vi "test resource blob.vi"(8 "error in (no error)":errorcluster) -> (0 "error out":errorcluster, 3 "body":string)   [LabVIEW 2020, in "MCP Server tests.lvlib"]
doc: "resources/read of a binary file (image/png) must return blob: the Base64 encoding of the exact bytes of the file, as a plain JSON string."
uses:
  MCP Server tests.lvlib
  <vilib>/JDP Science/JSONtext/Next JSON Value.vi
  <vilib>/JDP Science/JSONtext/String Subset.vi
  <vilib>/JDP Science/JSONtext/Parsing/Advance past next JSON Value (inlined COPY).vi
  <vilib>/JDP Science/JSONtext/Parsing/Advance past whitespace.vi
  <vilib>/JDP Science/JSONtext/Parsing/Advance past String.vi
  <vilib>/JDP Science/JSONtext/Parsing/Advance past Number.vi
  <vilib>/JDP Science/JSONtext/Parsing/Advance past Line Ending.vi
  <vilib>/JDP Science/JSONtext/Parsing/Parse Full Path or Item Name.vi
  <vilib>/JDP Science/JSONtext/Parsing/Advance past Array.vi
  <vilib>/JDP Science/JSONtext/Parsing/Advance past Object.vi
  <vilib>/JDP Science/JSONtext/support/Error Cluster From Code.vi
  <vilib>/JDP Science/JSONtext/Offset/Find Item Locations by Path.vi
  <vilib>/addons/_JKI Toolkits/Caraya/classes/Test/Test.lvclass
  <vilib>/JDP Science/JSONtext/JSONtext.lvlib
  <vilib>/JDP Science/JDP Science Common Utilities/Base64/Base64 Support.lvlib
  <vilib>/addons/_JKI Toolkits/Caraya/classes/Assert/Assert.lvclass
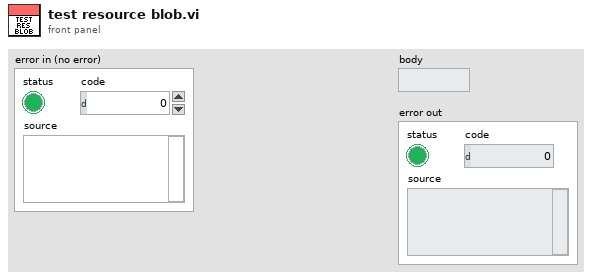
[diagram p1: front panel]
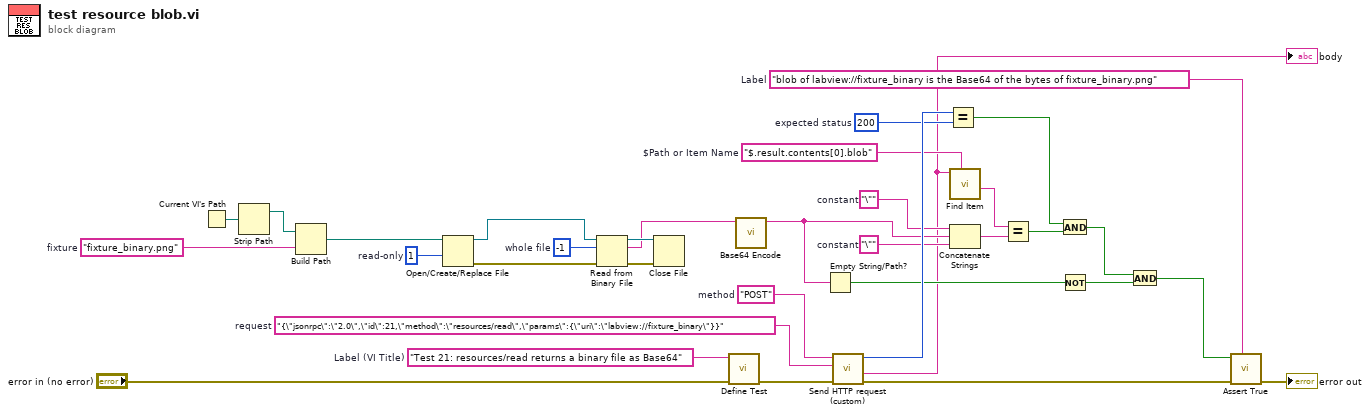
[diagram p0: block diagram]
diagram:
  w3 = "blob of labview://fixture_binary is the Base64 of the bytes of fixture_binary.png"  # Label
  w14 = "\""  # constant
  w15 = "\""  # constant
  w20 = -1  # whole file
  w22 = u32 1  # read-only
  w24 = "fixture_binary.png"  # fixture
  w27 = "$.result.contents[0].blob"  # $Path or Item Name
  w28 = 200  # expected status
  w31 = "{\"jsonrpc\":\"2.0\",\"id\":21,\"method\":\"resources/read\",\"params\":{\"uri\":\"labview://fixture_binary\"}}"  # request
  w32 = "POST"  # method
  w34 = "Test 21: resources/read returns a binary file as Base64"  # Label (VI Title)
  n1 = Current VI's Path() -> (path=w26:path)
  n2 = Strip Path(path=w26) -> (stripped path=w25:path)  [unwired: 1 out]
  n3 = Build Path(base path=w25, name or relative path=w24) -> (appended path=w23:path)
  n4 = Open/Create/Replace File(file path (use dialog)=w23, access (0:read/write)=w22) -> (refnum out=w21:refnum<file>, error out=w19:errorcluster)  [unwired: 4 in, 1 out]
  n5 = Read from Binary File(8:w19, 10:w20, 11:w21) -> (0:w17:errorcluster, 2:w16:string, 3:w18:refnum<file>)  [unwired: 3 in, 1 out]
  n6 = Close File(refnum=w18, error in=w17) -> ()  [unwired: 2 out]
  n7 = call <vilib>:"Define Test.vi"("error in (no error)"="error in (no error)", "Label (VI Title)"=w34) -> ("error out"=w30:errorcluster)  [unwired: 8 in, 1 out]
  n8 = call <vilib>:"Base64 Encode.vi"("String to Encode"=w16) -> ("Base64 Encoded"=w11:string)  [unwired: 10 in]
  n9 = Empty String/Path?(string/path=w11) -> (empty?=w10:bool)
  n10 = call "Send HTTP request (custom).vi"("error in (no error)"=w30, "request"=w31, "method"=w32) -> ("error out"=w4:errorcluster, "response"=w2:string, "status code"=w29:i32)  [unwired: 5 in, 1 out]
  "body" <- w2
  n11 = Equal?(x=w29, y=w28) -> (x = y?=w9:bool)
  n12 = call <vilib>:"Find Item.vi"("$Path or Item Name"=w27, "JSON"=w2) -> ("<JSON>"=w13:string)  [unwired: 6 in, 3 out]
  n13 = Concatenate Strings(w15, w11, w14) -> (w12:string)
  n14 = Equal?(x=w13, y=w12) -> (x = y?=w8:bool)
  n15 = And(x=w9, y=w8) -> (x .and. y?=w7:bool)
  n16 = Not(x=w10) -> (.not. x?=w6:bool)
  n17 = And(x=w7, y=w6) -> (x .and. y?=w5:bool)
  n18 = call <vilib>:"Assert True.vi"("Label"=w3, "error in (no error)"=w4, "True?"=w5) -> ("error out"=→"error out":errorcluster)  [unwired: 7 in, 1 out]
